vi "License.vi"   [LabVIEW 2021]
uses:
  SHELL32.DLL
panel:
  # "CalcExpress Toolkit\n[License]"
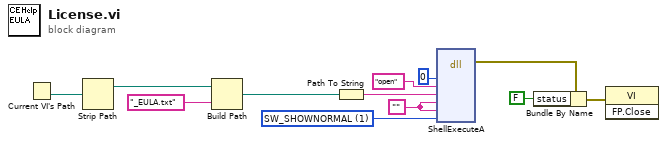
[diagram p0: block diagram]
diagram:
  w4 = 1 items=["SW_HIDE", "SW_SHOWNORMAL", "SW_SHOWMINIMIZED", "SW_SHOWMAXIMIZED", "SW_SHOWNOACTIVE", "SW_SHOW", "SW_MINIMIZE", "SW_SHOWMINNOACTIVE", "SW_SHOWNA", "SW_RESTORE", "SW_SHOWDEFAULT", "SW_FORCEMINIMIZE"] ("show (normal)")
  w9 = ""
  n1 = Current VI's Path() -> (path=w12:path)
  n2 = Strip Path(path=w12) -> (stripped path=w11:path)  [unwired: 1 out]
  n3 = Build Path(base path=w11, name or relative path="_EULA.txt") -> (appended path=w5:path)
  n4 = Path To String(path=w5) -> (string=w7:string)
  n5 = dll-call lib="SHELL32.DLL" fn="ShellExecuteA"("hWnd"=0, "Operation"="open", "File"=w7, "Parameters"=w9, "DefaultDir"=w9, "ShowCmd"=w4) -> (error out=w3:errorcluster)  [unwired: 10 in, 1 out]
  n6 = Bundle By Name(cluster=w3, "status"=FALSE) -> (w2:errorcluster)
  n7 = invoke class="VI" method="FP.Close"(error in=w2) -> ()  [unwired: 2 in, 3 out]
